vi "Create.vi"(7 "Registry Name":string="_default_registry", 8 "error in (no error)":errorcluster, 9 "Auto-Register? (T)":bool=TRUE, 11 "Volumes":path[](array[path])) -> (0 "error out":errorcluster, 3 "Disk Collector out":refnum<class "Disk Collector.lvclass">)   [LabVIEW 2020, in "Disk Collector.lvclass"]
uses:
  Disk Collector.lvclass
  C:/Github-locals/PromVIEW/src/collector/collectable/Collectable.lvclass
  Disk Collector.lvclass/Disk Collector.ctl
  src/metrics/gauge/Gauge.lvclass
  C:/Github-locals/PromVIEW/src/metrics/metric/Metric.lvclass
  src/registry/session/Registry Session.lvclass
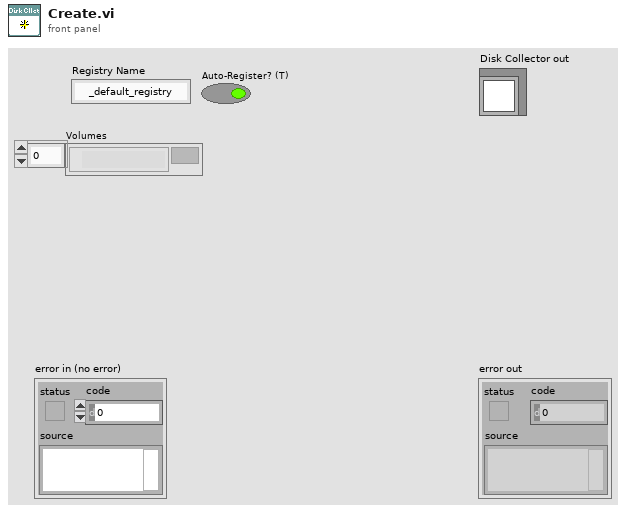
[diagram p1: front panel]
types:
  T1 = typedef "Registry.lvlib/Registry Session.lvclass/Session Handle.ctl" = refnum<data-value>
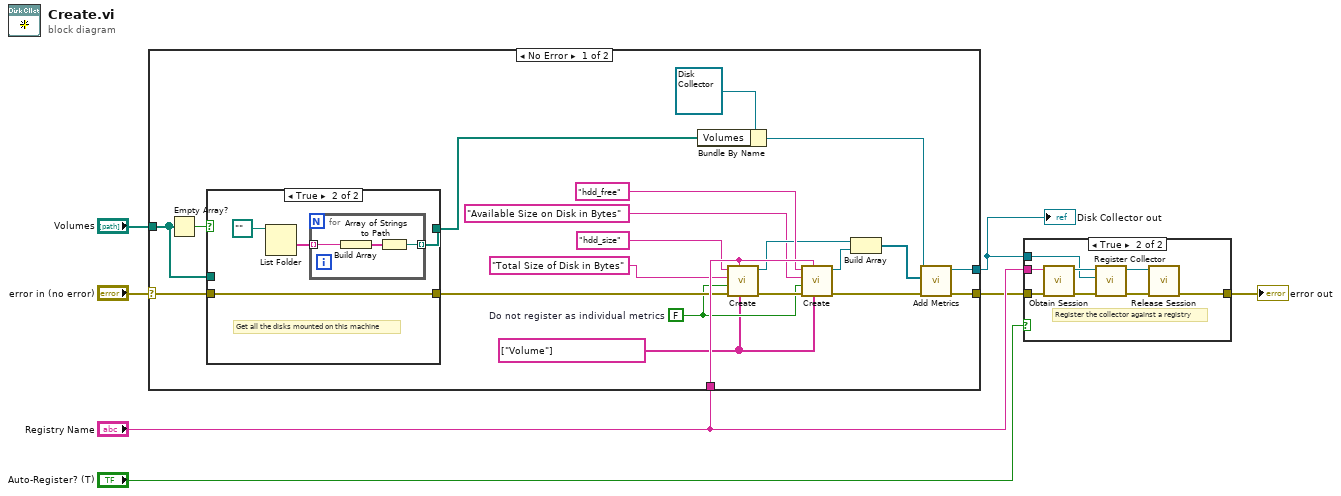
[diagram p0: block diagram]
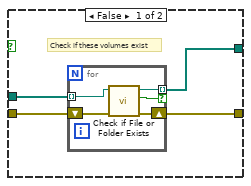
[diagram p2: hidden frame]
diagram:
  n1 = case shown="No Error" "error in (no error)" {
    selector: "error in (no error)" -> [w25 w45]
    tunnel: [w20 w45] -> w4
    tunnel: [w22 _] -> w3
    tunnel: "Volumes" -> [w26 _]
    tunnel: "Registry Name" -> [w19 _]
    frame No Error {
      w8 = string[] ["Volume"] ("Label Names")
      w9 = FALSE  # Do not register as individual metrics
      n2 = Empty Array?(array=w26) -> (empty?=w27:bool)
      n3 = case shown="True" w27 {
        tunnel: w26 -> [w32 _]
        tunnel: [w31 w39] -> w23
        tunnel: w25 -> [w30 w38]
        tunnel: [w29 w38] -> w17
        frame False {
          # "Check if these volumes exist"
          n4 = for {
            tunnel: w32 -> [w37] mode=indexing
            tunnel: [w36] -> w31 mode=indexing if=w35
            shift-right: [w33] -> w29
            shift-left: w30 -> [w34]
            n5 = call <vilib>:"Check if File or Folder Exists.vi"("error in (no error)"=w34, "path"=w37) -> ("error out"=w33:errorcluster, "file or folder exists?"=w35:bool, "dup path"=w36:path)  [unwired: 7 in]
          }
        }
        frame True {
          # "Get all the disks mounted on this machine"
          n6 = List Folder(path=path "") -> (folder names=w40:string[])  [unwired: 3 in, 3 out]
          n7 = for {
            tunnel: w40 -> [w43] mode=indexing
            tunnel: [w44] -> w39 mode=indexing
            n8 = Build Array(w43) -> (w42:string[])
            n9 = Array of Strings to Path(0:w42) -> (2:w44:path)  [unwired: 1 in]
          }
        }
      }
      n10 = Bundle By Name(cluster=refnum<class "Disk Collector.lvclass"> refnum ("Disk Collector in"), "Volumes"=w23) -> (w28:refnum<class "Disk Collector.lvclass">)
      n11 = call "Create.vi"("Label Names"=w8, "Registry Name"=w19, "error in (no error)"=w17, "Auto-register?"=w9, "Description"="Total Size of Disk in Bytes" ("format string"), "Metric Name"="hdd_size" ("format string")) -> ("error out"=w14:errorcluster, "Gauge Ref"=w12:refnum<data-value>)  [unwired: 4 in]
      n12 = call "Create.vi"("Label Names"=w8, "Registry Name"=w19, "error in (no error)"=w14, "Auto-register?"=w9, "Description"="Available Size on Disk in Bytes" ("format string"), "Metric Name"="hdd_free" ("format string")) -> ("error out"=w18:errorcluster, "Gauge Ref"=w13:refnum<data-value>)  [unwired: 4 in]
      n13 = Build Array(w12, w13) -> (w21:refnum<data-value>[])
      n14 = call-dynamic "Add Metrics.vi"("error in (no error)"=w18, "Metrics"=w21, "Default Collector in"=w28) -> ("error out"=w20:errorcluster, "Default Collector out"=w22:refnum<class "Disk Collector.lvclass">)  [unwired: 7 in]
    }
    frame Error {
    }
  }
  "Disk Collector out" <- w3
  n15 = case shown="True" "Auto-Register? (T)" {
    tunnel: "Registry Name" -> [_ w54]
    tunnel: w4 -> [w46 w53]
    tunnel: w3 -> [_ w50]
    tunnel: [w46 w47] -> w1
    frame False {
    }
    frame True {
      # "Register the collector against a registry"
      n16 = call "Obtain Session.vi"("error in (no error)"=w53, "Session  Name ()"=w54) -> ("error out"=w52:errorcluster, "Session Handle"=w51:T1)  [unwired: 8 in]
      n17 = call "Register Collector.vi"("error in (no error)"=w52, "Collector"=w50, "Session Handle in"=w51) -> ("error out"=w49:errorcluster, "Session Handle out"=w48:T1)  [unwired: 7 in]
      n18 = call "Release Session.vi"("error in (no error)"=w49, "Session Handle"=w48) -> ("error out"=w47:errorcluster)  [unwired: 9 in]
    }
  }
  "error out" <- w1
